vi "错误输入.vi"(9 "source":string, 10 "code(0)":i32, 11 "status(T)":bool=TRUE) -> (0 "error out":errorcluster caption="错误输出")   [LabVIEW 2025]
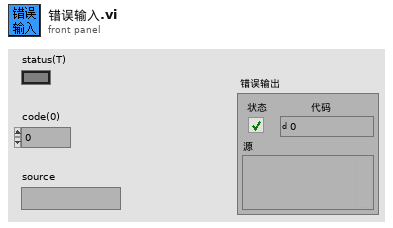
[diagram p1: front panel]
types:
  T1 = cluster{"status(T)":bool, "code(0)":i32, "source":string}
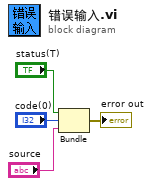
[diagram p0: block diagram]
diagram:
  n1 = Bundle("status(T)"="status(T)", "code(0)"="code(0)", "source"="source") -> (→"error out":T1)  [unwired: 1 in]
